vi "MAIZE Vacuum Console.vi"() -> ()   [LabVIEW 2025]
doc: "MAIZE vacuum rack. Four read-only valve lamps and the local controller interlocks."
panel:
  in  "End session":bool
  out "Cryo gate valve":picture
  out "Turbo gate valve":picture
  out "Let-up valve":picture
  out "Roughing valve":picture
  out "Latched faults":string
  out "Active interlocks":string
  out "Opening outputs":string
  out "Chamber pressure":string
  out "Operating state":string
  out "Controller link":string
  # "MAIZE     /     Vacuum control"
  # "Levers follow the physical toggles"
  # "OPEN   Red        CLOSED   Green        UNKNOWN   Grey"
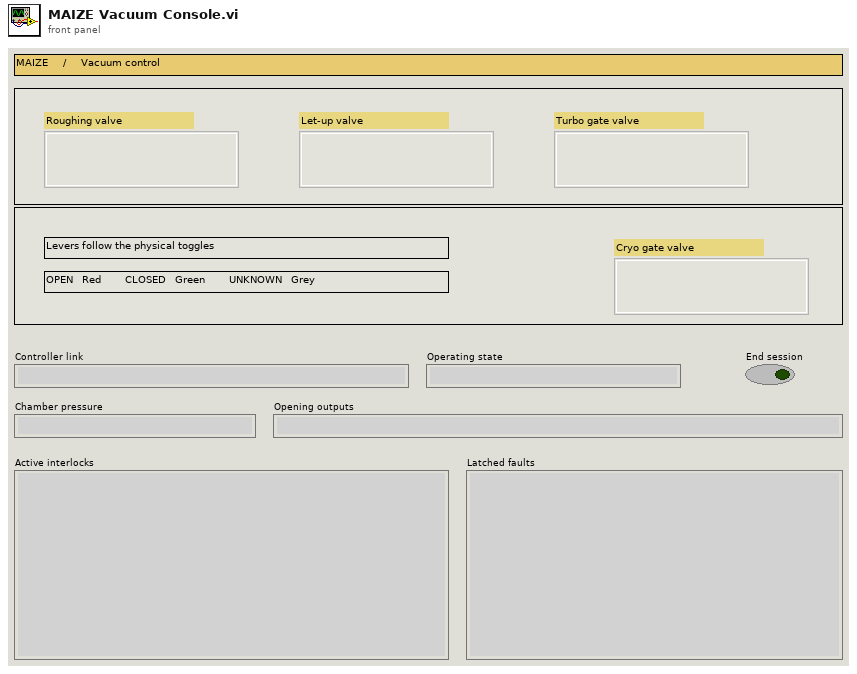
[diagram p1: front panel]
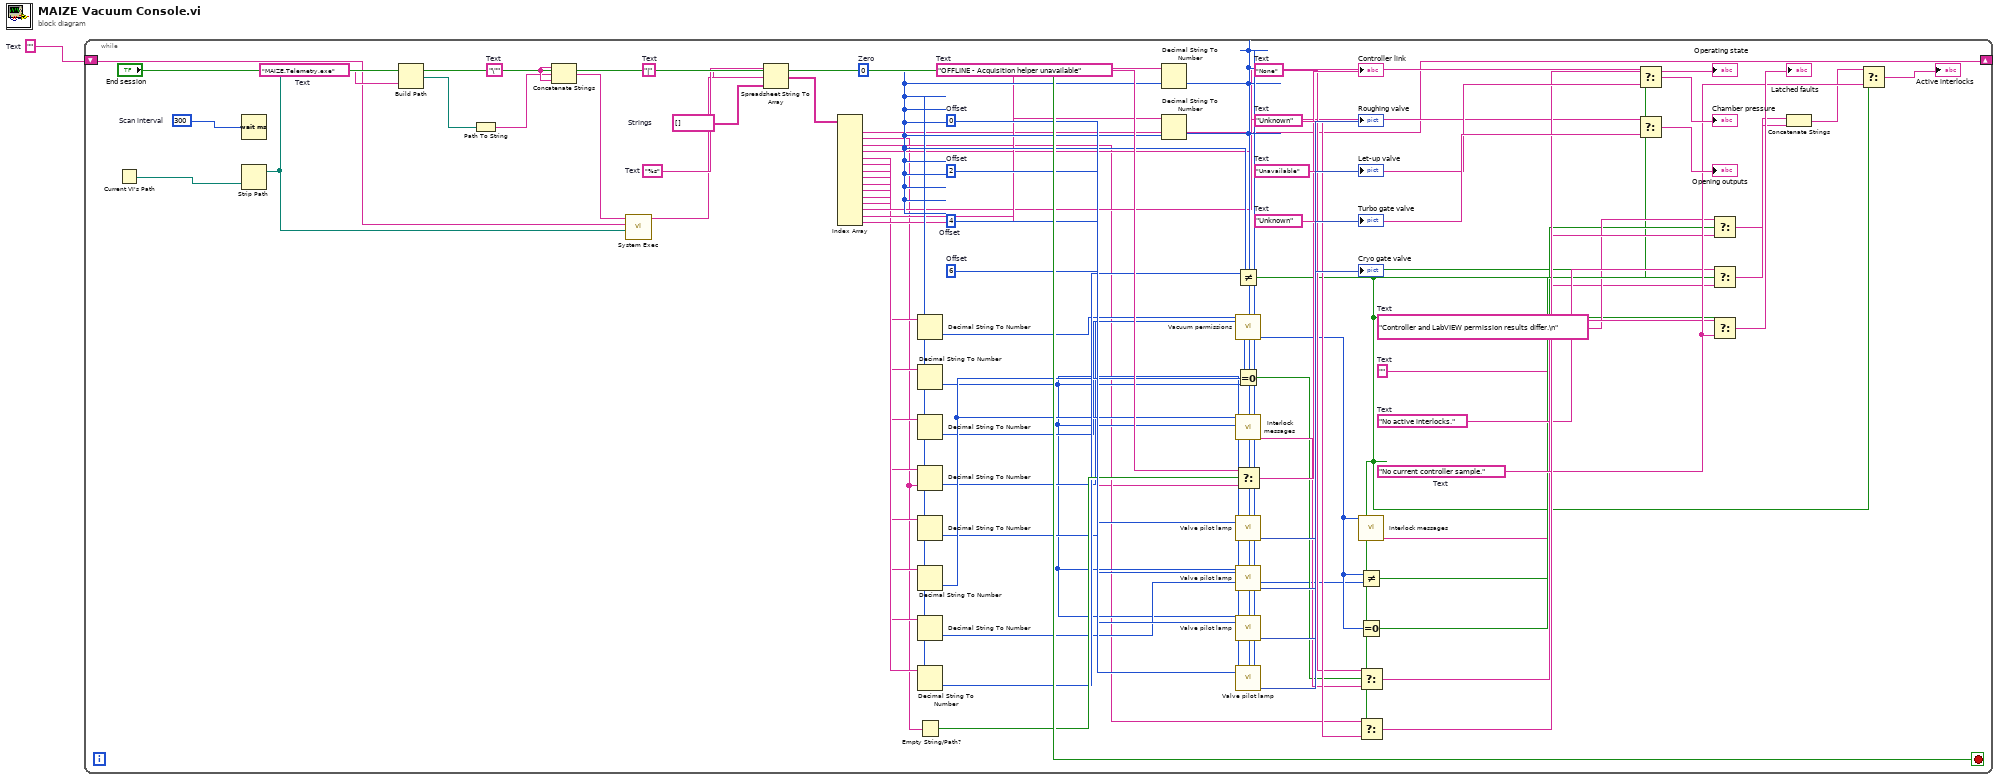
[diagram p0: block diagram]
diagram:
  w1 = ""  # Text
  n1 = while {
    shift-right: [w3] -> _
    shift-left: w1 -> [w2]
    stop <- "End session" stop-if-true
    w76 = u32 300  # Scan interval
    w74 = u32 6  # Offset
    w72 = u32 4  # Offset
    w70 = u32 2  # Offset
    w68 = u32 0  # Offset
    w62 = "Unknown"  # Text
    w60 = "Unavailable"  # Text
    w58 = "Unknown"  # Text
    w56 = "OFFLINE - Acquisition helper unavailable"  # Text
    w54 = "No current controller sample."  # Text
    w51 = "None"  # Text
    w47 = "No active interlocks."  # Text
    w44 = ""  # Text
    w43 = "Controller and LabVIEW permission results differ.\n"  # Text
    w30 = u32 0  # Zero
    w14 = "%s"  # Text
    w13 = string[] []  # Strings
    w12 = "|"  # Text
    w9 = "\""  # Text
    w6 = "MAIZE.Telemetry.exe"  # Text
    n2 = Current VI's Path() -> (path=w4:path)
    n3 = Wait (ms)(milliseconds to wait=w76) -> ()  [unwired: 1 out]
    n4 = Strip Path(path=w4) -> (stripped path=w5:path)  [unwired: 1 out]
    n5 = Build Path(base path=w5, name or relative path=w6) -> (appended path=w7:path)
    n6 = Path To String(path=w7) -> (string=w8:string)
    n7 = Concatenate Strings(w9, w8, w9) -> (w10:string)
    n8 = call <vilib>:"System Exec.vi"("working directory"=w5, "standard input"=w2, "command line"=w10) -> ("standard output"=w11:string)  [unwired: 5 in, 3 out]
    n9 = Spreadsheet String To Array(delimiter (Tab)=w12, format string=w14, spreadsheet string=w11, array type (2D Dbl)=w13) -> (array=w15:string[])
    n10 = Index Array(array=w15) -> (element #1=w3:string, element #2=w16:string, element #3=w17:string, element #4=w18:string, element #5=w19:string, element #6=w20:string, element #7=w21:string, element #8=w22:string, element #9=w23:string, element #10=w24:string, element #11=w25:string, element #12=w26:string, element #13=w27:string, element #14=w28:string, element #15=w29:string)  [unwired: 15 in]
    n11 = Decimal String To Number(string=w19, default (0L)=w30) -> (number=w31:u32)  [unwired: 1 in, 1 out]
    n12 = Decimal String To Number(string=w20, default (0L)=w30) -> (number=w32:u32)  [unwired: 1 in, 1 out]
    n13 = Decimal String To Number(string=w21, default (0L)=w30) -> (number=w33:u32)  [unwired: 1 in, 1 out]
    n14 = Decimal String To Number(string=w22, default (0L)=w30) -> (number=w34:u32)  [unwired: 1 in, 1 out]
    n15 = Decimal String To Number(string=w23, default (0L)=w30) -> (number=w35:u32)  [unwired: 1 in, 1 out]
    n16 = Decimal String To Number(string=w24, default (0L)=w30) -> (number=w36:u32)  [unwired: 1 in, 1 out]
    n17 = Decimal String To Number(string=w25, default (0L)=w30) -> (number=w37:u32)  [unwired: 1 in, 1 out]
    n18 = Decimal String To Number(string=w26, default (0L)=w30) -> (number=w38:u32)  [unwired: 1 in, 1 out]
    n19 = Empty String/Path?(string/path=w16) -> (empty?=w55:bool)
    n20 = Decimal String To Number(string=w28, default (0L)=w30) -> (number=w66:u32)  [unwired: 1 in, 1 out]
    n21 = Decimal String To Number(string=w29, default (0L)=w30) -> (number=w67:u32)  [unwired: 1 in, 1 out]
    n22 = Not Equal?(x=w38, y=w30) -> (x != y?=w39:bool)
    n23 = call "Vacuum permissions.vi"("attempt"=w31, "pos"=w32, "status"=w33, "site"=w34, "events"=w35) -> ("alarms"=w40:u32)  [unwired: 10 in]
    n24 = Equal To 0?(x=w36) -> (x = 0?=w50:bool)
    n25 = call "Interlock messages.vi"("Fault bits"=w36) -> ("Messages"=w52:string)  [unwired: 14 in]
    n26 = Select(t=w56, s=w55, f=w16) -> (s? t:f=→"Controller link":string)
    n27 = call "Valve pilot lamp.vi"("Position word"=w32, "Bit offset"=w68, "Physical selectors"=w66, "Selector quality"=w67) -> ("Lamp"=→"Roughing valve":picture)  [unwired: 11 in]
    n28 = call "Valve pilot lamp.vi"("Position word"=w32, "Bit offset"=w70, "Physical selectors"=w66, "Selector quality"=w67) -> ("Lamp"=→"Let-up valve":picture)  [unwired: 11 in]
    n29 = call "Valve pilot lamp.vi"("Position word"=w32, "Bit offset"=w72, "Physical selectors"=w66, "Selector quality"=w67) -> ("Lamp"=→"Turbo gate valve":picture)  [unwired: 11 in]
    n30 = call "Valve pilot lamp.vi"("Position word"=w32, "Bit offset"=w74, "Physical selectors"=w66, "Selector quality"=w67) -> ("Lamp"=→"Cryo gate valve":picture)  [unwired: 11 in]
    n31 = call "Interlock messages.vi"("Fault bits"=w40) -> ("Messages"=w41:string)  [unwired: 14 in]
    n32 = Not Equal?(x=w40, y=w37) -> (x != y?=w42:bool)
    n33 = Equal To 0?(x=w40) -> (x = 0?=w46:bool)
    n34 = Select(t=w51, s=w50, f=w52) -> (s? t:f=w53:string)
    n35 = Select(t=w17, s=w39, f=w58) -> (s? t:f=→"Operating state":string)
    n36 = Select(t=w18, s=w39, f=w60) -> (s? t:f=→"Chamber pressure":string)
    n37 = Select(t=w27, s=w39, f=w62) -> (s? t:f=→"Opening outputs":string)
    n38 = Select(t=w43, s=w42, f=w44) -> (s? t:f=w45:string)
    n39 = Select(t=w47, s=w46, f=w41) -> (s? t:f=w48:string)
    n40 = Select(t=w53, s=w39, f=w54) -> (s? t:f=→"Latched faults":string)
    n41 = Concatenate Strings(w45, w48) -> (w49:string)
    n42 = Select(t=w49, s=w39, f=w54) -> (s? t:f=→"Active interlocks":string)
  }
